vi "Power Supply.vi"() -> ()   [LabVIEW 2026]
uses:
  <vilib>/numeric/Random Number (Range) DBL.vi
panel:
  out "Connected?":bool
  in  "Voltage Setpoint":dbl(knob) scale=0.0..20.0
  out "Stopped?":bool
  in  "stop":bool
  out "IP Address":string
  in  "Enable?":bool
  out "Power Supply Current":dbl(knob) scale=0.0..5.0
  out "Power Supply Voltage":dbl(knob) scale=0.0..20.0
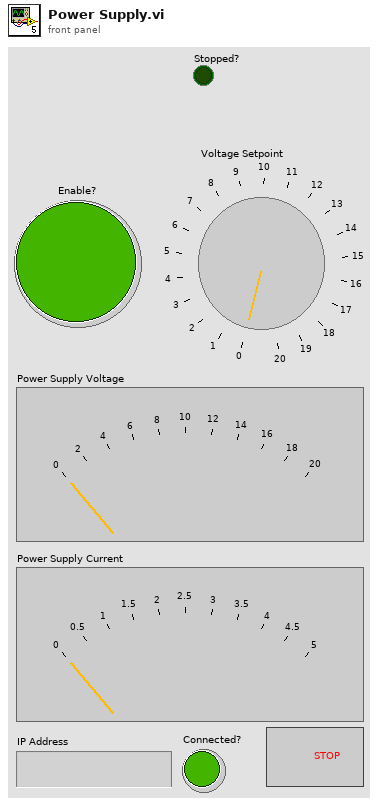
[diagram p1: front panel]
types:
  T1 = enum16{"Standard", "Buffered", "CRLF", "Immediate"}
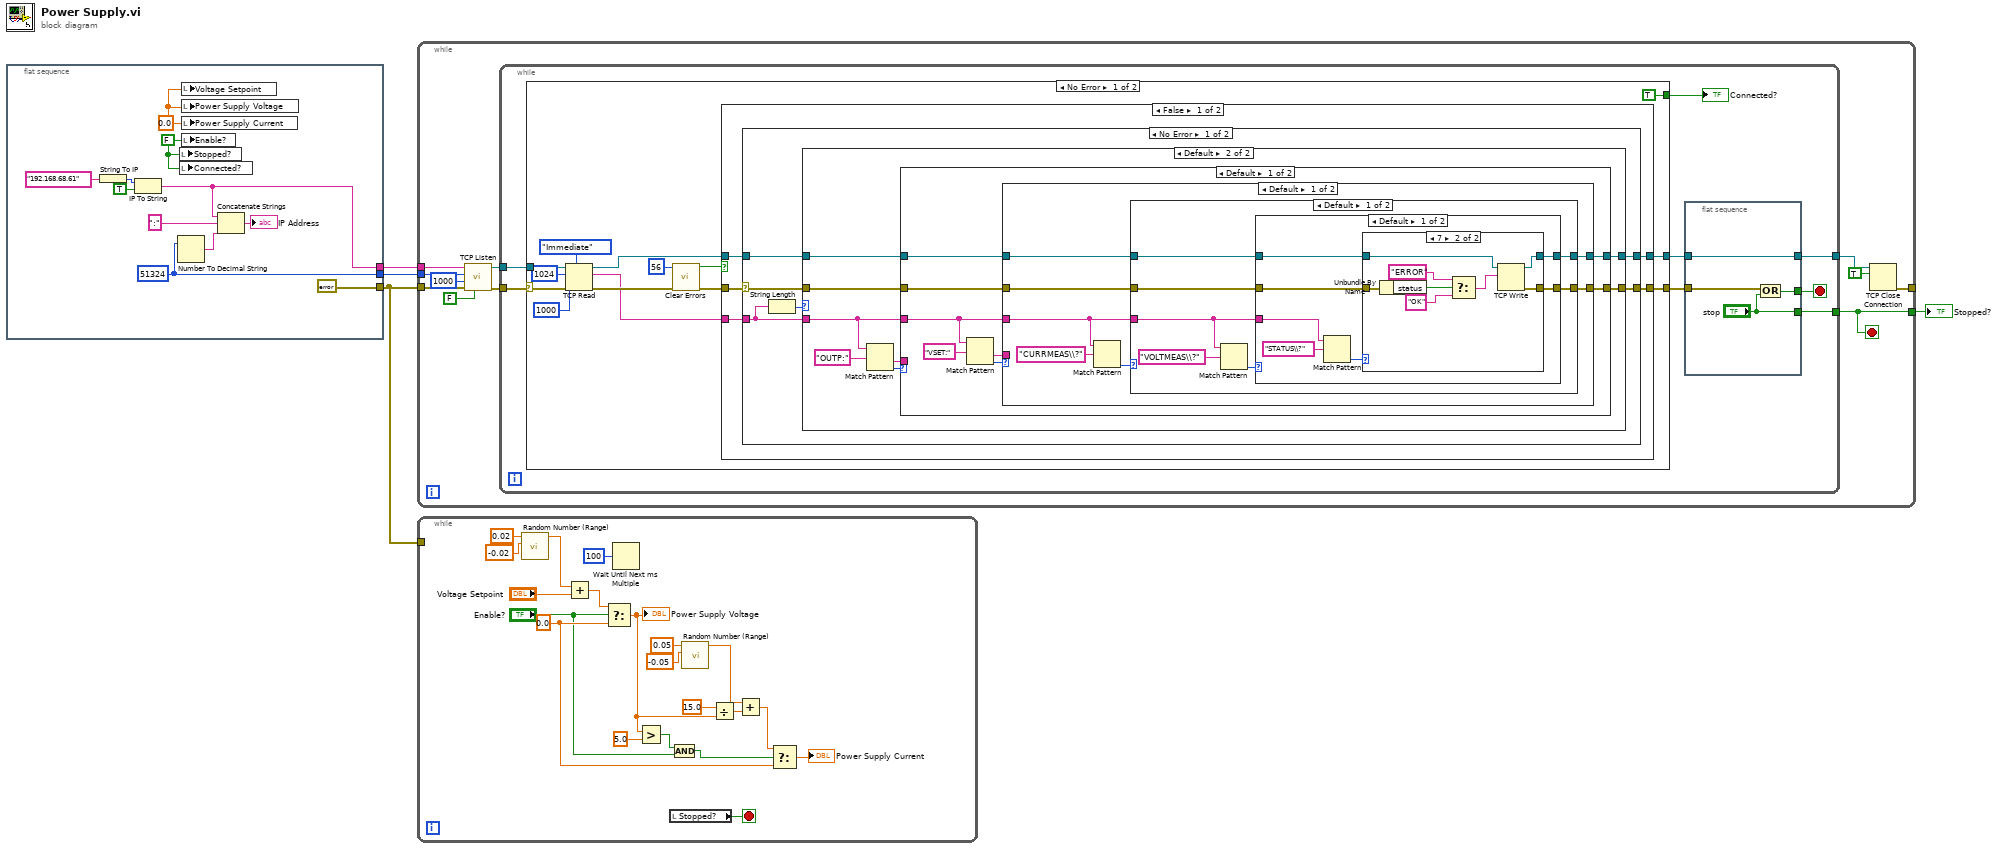
[diagram p0: block diagram]
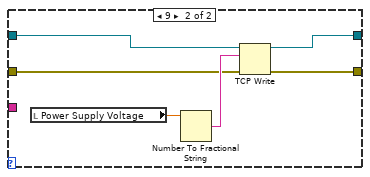
[diagram p4: hidden frame]
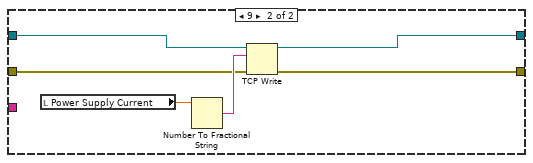
[diagram p5: hidden frame]
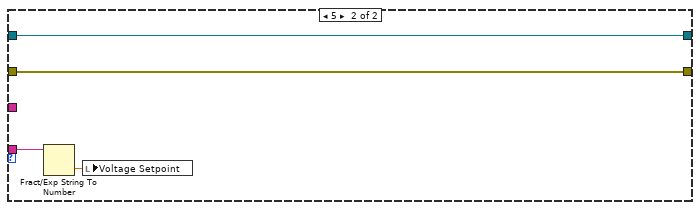
[diagram p6: hidden frame]
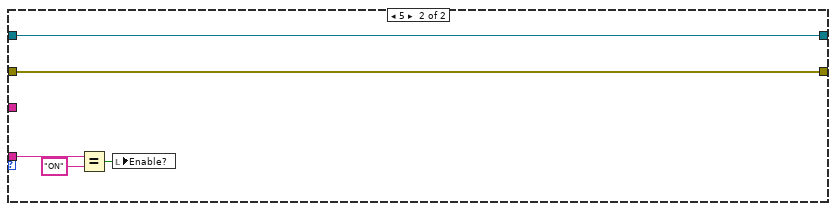
[diagram p7: hidden frame]
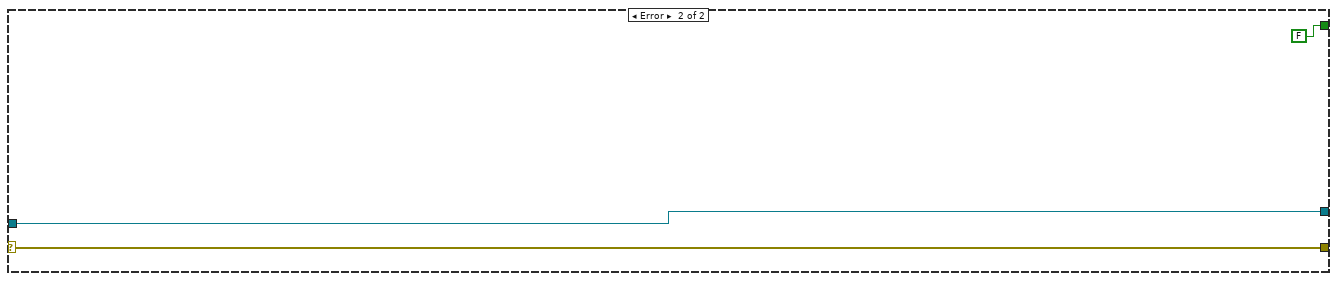
[diagram p10: hidden frame]
diagram:
  n1 = flat-sequence {
    tunnel: [w13] -> w4
    tunnel: [w11] -> w3
    tunnel: [errorcluster {"status"=FALSE, "code"=0, "source"=""} ("error in (no error)")] -> w1
    frame #0 {
      w9 = 0.0 ("Power Supply Current")
      w6 = FALSE ("Enable?")
      w13 = u16 51324 ("port")
      n2 = String To IP(1:"192.168.68.61" ("name")) -> (0:w8:u32)
      n3 = IP To String(1:TRUE ("dot notation? (F)"), 2:w8) -> (0:w11:string)
      n4 = Number To Decimal String(number=w13) -> (decimal integer string=w12:string)  [unwired: 1 in]
      n5 = local write "Stopped?"(w6) -> ()
      n6 = local write "Connected?"(w6) -> ()
      n7 = local write "Voltage Setpoint"(w9) -> ()
      n8 = local write "Power Supply Voltage"(w9) -> ()
      n9 = local write "Power Supply Current"(w9) -> ()
      n10 = local write "Enable?"(w6) -> ()
      n11 = Concatenate Strings(w11, ":" ("string"), w12) -> (→"IP Address":string)
    }
  }
  n12 = while {
    tunnel: w4 -> [w26]
    tunnel: w3 -> [w25]
    tunnel: [w20] -> w2
    tunnel: w1 -> [w22]
    tunnel: [w17] -> _
    stop <- w20 stop-if-true
    n13 = call <vilib>:"TCP Listen.vi"("resolve remote address (T)"=FALSE, "error in (no error)"=w22, "timeout ms (wait forever: -1)"=1000, "port"=w26, "service name"=w25) -> ("error out"=w23:errorcluster, "connection ID"=w24:refnum<k5>)  [unwired: 2 in, 3 out]
    n14 = while {
      tunnel: w24 -> [w34]
      tunnel: w23 -> [w31]
      tunnel: [w30] -> w20
      tunnel: [w28] -> w19
      stop <- w32 stop-if-true
      n15 = case shown="No Error" w31 {
        selector: w31 -> [w36 w136]
        tunnel: w34 -> [w48 w135]
        tunnel: [w38 w136] -> w33
        tunnel: [w37 w135] -> w29
        tunnel: [TRUE FALSE] -> w27
        frame No Error {
          n16 = TCP Read(connection ID=w48, bytes to read=1024, error in (no error)=w36, 7:T1."Immediate" ("mode (standard)"), 9:1000 ("timeout ms (25000)")) -> (connection ID out=w39:refnum<k5>, data out=w41:string, error out=w45:errorcluster)
          n17 = call <vilib>:"Clear Errors.vi"("error in (no error)"=w45, "specific error code to clear (0: all)"=56) -> ("error out"=w42:errorcluster, "specific error cleared?"=w43:bool)  [unwired: 4 in]
          n18 = case shown="False" w43 {
            tunnel: w42 -> [w53 w133]
            tunnel: w41 -> [w52 _]
            tunnel: w39 -> [w51 w132]
            tunnel: [w50 w133] -> w38
            tunnel: [w49 w132] -> w37
            frame False {
              n19 = case shown="No Error" w53 {
                selector: w53 -> [w58 w131]
                tunnel: w52 -> [w56 _]
                tunnel: w51 -> [w57 w130]
                tunnel: [w55 w131] -> w50
                tunnel: [w54 w130] -> w49
                frame No Error {
                  n20 = String Length(string=w56) -> (length=w59:i32)
                  n21 = case shown="Default" w59 {
                    tunnel: w58 -> [w61 w64]
                    tunnel: w56 -> [_ w66]
                    tunnel: w57 -> [w60 w65]
                    tunnel: [w61 w63] -> w55
                    tunnel: [w60 w62] -> w54
                    frame 0 {
                    }
                    frame Default {
                      n22 = Match Pattern(string=w66, regular expression="OUTP:") -> (after substring=w67:string, offset past match=w68:i32)  [unwired: 1 in, 2 out]
                      n23 = case shown="Default" w68 {
                        tunnel: w67 -> [_ w129]
                        tunnel: w66 -> [w74 _]
                        tunnel: w65 -> [w73 w125]
                        tunnel: [w72 w126] -> w63
                        tunnel: w64 -> [w71 w126]
                        tunnel: [w70 w125] -> w62
                        frame Default {
                          n24 = Match Pattern(string=w74, regular expression="VSET:") -> (after substring=w77:string, offset past match=w76:i32)  [unwired: 1 in, 2 out]
                          n25 = case shown="Default" w76 {
                            tunnel: w77 -> [_ w124]
                            tunnel: w74 -> [w81 _]
                            tunnel: w73 -> [w83 w121]
                            tunnel: [w80 w122] -> w72
                            tunnel: w71 -> [w79 w122]
                            tunnel: [w78 w121] -> w70
                            frame Default {
                              n26 = Match Pattern(string=w81, regular expression="CURRMEAS\\?") -> (offset past match=w82:i32)  [unwired: 1 in, 3 out]
                              n27 = case shown="Default" w82 {
                                tunnel: w83 -> [w89 w118]
                                tunnel: w81 -> [w87 _]
                                tunnel: [w88 w116] -> w80
                                tunnel: w79 -> [w86 w117]
                                tunnel: [w85 w115] -> w78
                                frame Default {
                                n28 = Match Pattern(string=w87, regular expression="VOLTMEAS\\?") -> (offset past match=w90:i32)  [unwired: 1 in, 3 out]
                                n29 = case shown="Default" w90 {
                                tunnel: w89 -> [w95 w112]
                                tunnel: [w94 w111] -> w88
                                tunnel: w87 -> [w97 _]
                                tunnel: w86 -> [w96 w110]
                                tunnel: [w92 w109] -> w85
                                frame Default {
                                n30 = Match Pattern(string=w97, regular expression="STATUS\\?") -> (offset past match=w93:i32)  [unwired: 1 in, 3 out]
                                n31 = case shown="7" w93 {
                                tunnel: w96 -> [w100 w108]
                                tunnel: w95 -> [w99 w103]
                                tunnel: [w100 w102] -> w94
                                tunnel: [w99 w101] -> w92
                                frame 0, Default {
                                }
                                frame 7 {
                                n32 = Unbundle By Name(w108) -> ("status"=w107:bool)
                                n33 = Select(t="ERROR", s=w107, f="OK") -> (s? t:f=w104:string)
                                n34 = TCP Write(connection ID=w103, data in=w104) -> (connection ID out=w101:refnum<k5>, error out=w102:errorcluster)  [unwired: 2 in, 1 out]
                                }
                                }
                                }
                                frame 9 {
                                n35 = local read "Power Supply Voltage"() -> (w113:dbl)
                                n36 = Number To Fractional String(number=w113) -> (F-format string=w114:string)  [unwired: 3 in]
                                n37 = TCP Write(connection ID=w112, data in=w114, error in (no error)=w110) -> (connection ID out=w109:refnum<k5>, error out=w111:errorcluster)  [unwired: 1 in, 1 out]
                                }
                                }
                                }
                                frame 9 {
                                n38 = local read "Power Supply Current"() -> (w119:dbl)
                                n39 = Number To Fractional String(number=w119) -> (F-format string=w120:string)  [unwired: 3 in]
                                n40 = TCP Write(connection ID=w118, data in=w120, error in (no error)=w117) -> (connection ID out=w115:refnum<k5>, error out=w116:errorcluster)  [unwired: 1 in, 1 out]
                                }
                              }
                            }
                            frame 5 {
                              n41 = Fract/Exp String To Number(string=w124) -> (number=w123:dbl)  [unwired: 3 in, 1 out]
                              n42 = local write "Voltage Setpoint"(w123) -> ()
                            }
                          }
                        }
                        frame 5 {
                          n43 = Equal?(x=w129, y="ON") -> (x = y?=w127:bool)
                          n44 = local write "Enable?"(w127) -> ()
                        }
                      }
                    }
                  }
                }
                frame Error {
                }
              }
            }
            frame True {
            }
          }
        }
        frame Error {
        }
      }
      "Connected?" <- w27
      n45 = flat-sequence {
        tunnel: w33 -> [w139]
        tunnel: [w140] -> w32
        tunnel: ["stop"] -> w30
        tunnel: w29 -> [w137]
        tunnel: [w137] -> w28
        frame #0 {
          n46 = Compound Arithmetic op=OR(w139, "stop") -> (w140:bool)
        }
      }
    }
    n47 = TCP Close Connection(connection ID=w19, abort (F)=TRUE) -> (error out=w17:errorcluster)  [unwired: 1 in, 1 out]
  }
  "Stopped?" <- w2
  n48 = while {
    tunnel: w1 -> [_]
    stop <- w152 stop-if-true
    w155 = 0.0 ("f")
    n49 = call-poly <vilib>:"Random Number (Range).vi"("lower bound (0)"=-0.02 ("upper bound (100)"), "upper bound (100)"=0.02) -> ("number"=w158:dbl)  [unwired: 9 in]
    n50 = Add(x=w158, y="Voltage Setpoint") -> (x+y=w157:dbl)
    n51 = Select(t=w157, s="Enable?", f=w155) -> (s? t:f=w144:dbl)
    "Power Supply Voltage" <- w144
    n52 = Wait Until Next ms Multiple(millisecond multiple=u32 100) -> ()  [unwired: 1 out]
    n53 = Greater?(x=w144, y=5.0) -> (0:w148:bool)
    n54 = local read "Stopped?"() -> (w152:bool)
    n55 = And(x=w148, y="Enable?") -> (x .and. y?=w146:bool)
    n56 = call-poly <vilib>:"Random Number (Range).vi"("lower bound (0)"=-0.05 ("upper bound (100)"), "upper bound (100)"=0.05) -> ("number"=w142:dbl)  [unwired: 9 in]
    n57 = Divide(x=15.0, y=w144) -> (x/y=w143:dbl)
    n58 = Add(x=w142, y=w143) -> (x+y=w141:dbl)
    n59 = Select(t=w141, s=w146, f=w155) -> (s? t:f=→"Power Supply Current":dbl)
  }
